vi "Write Modbus_Master.lvclass.vi"(8 "error in (no error)":errorcluster, 10 "Modbus_Master.lvclass":refnum<class "Modbus_Master.lvclass">, 11 "Modbus_AI in":refnum<class "Modbus_AI.lvclass">) -> (0 "error out":errorcluster, 3 "Modbus_AI out":refnum<class "Modbus_AI.lvclass">)   [LabVIEW 2021, in "Modbus_AI.lvclass"]
uses:
  Modbus_AI.lvclass
  Modbus_Master/Modbus_Master.lvclass
  Modbus_AI.lvclass/Modbus_AI.ctl
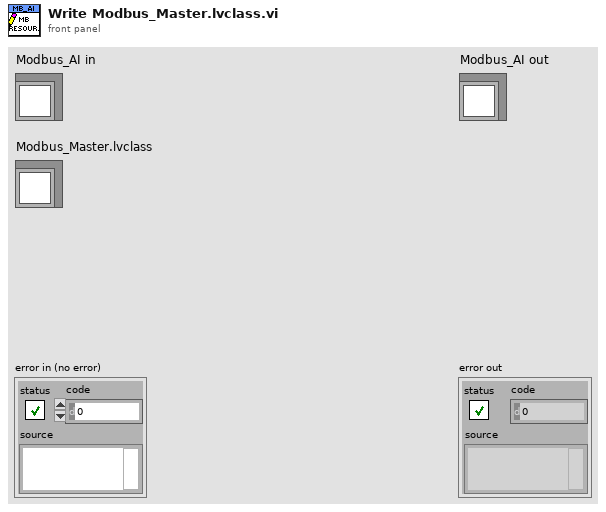
[diagram p1: front panel]
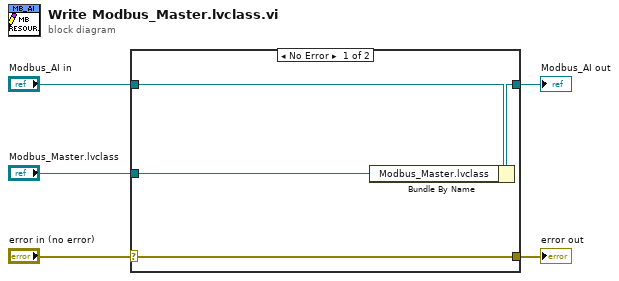
[diagram p0: block diagram]
diagram:
  n1 = case shown="No Error" "error in (no error)" {
    selector: "error in (no error)" -> [w9 w10]
    tunnel: [w9 w10] -> w4
    tunnel: [w7 w11] -> w2
    tunnel: "Modbus_AI in" -> [w8 w11]
    tunnel: "Modbus_Master.lvclass" -> [w6 _]
    frame No Error {
      n2 = Bundle By Name(cluster=w8, "Modbus_Master.lvclass"=w6) -> (w7:refnum<class "Modbus_AI.lvclass">)
    }
    frame Error {
    }
  }
  "error out" <- w4
  "Modbus_AI out" <- w2
